vi "Receive Message.vi"(8 "error in (no error)":errorcluster, 11 "SPARC4_GEI in":refnum<class "S4GEI.lvclass">) -> (0 "error out":errorcluster, 3 "SPARC4_GEI out":refnum<class "S4GEI.lvclass">)   [LabVIEW 2018, in "S4GEI.lvclass"]
uses:
  S4GEI.lvclass
  S4GEI.lvclass/S4GEI.ctl
  Channel GUI/Channel.lvclass
  RxTx/RxTx.lvclass
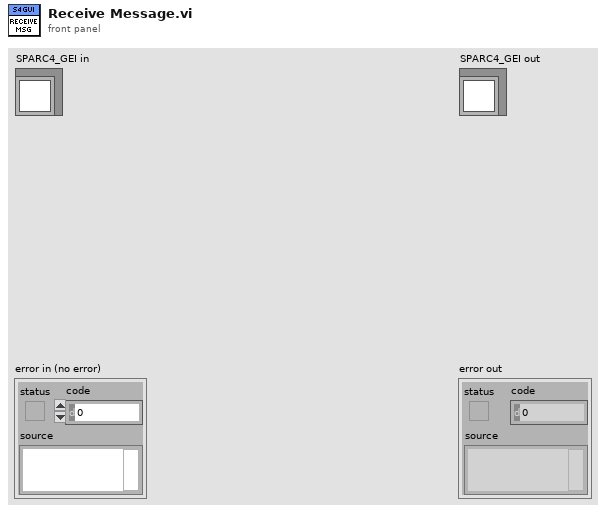
[diagram p1: front panel]
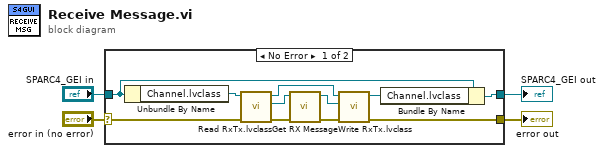
[diagram p0: block diagram]
diagram:
  n1 = case shown="No Error" "error in (no error)" {
    selector: "error in (no error)" -> [w12 w17]
    tunnel: [w10 w17] -> w3
    tunnel: [w14 w16] -> w1
    tunnel: "SPARC4_GEI in" -> [w15 w16]
    frame No Error {
      n2 = Unbundle By Name(w15) -> ("Channel.lvclass"=w13:refnum<class "Channel.lvclass">)
      n3 = call "Read RxTx.lvclass.vi"("error in (no error)"=w12, "Channel GUI in"=w13) -> ("error out"=w6:errorcluster, "RxTx.lvclass"=w9:refnum<class "RxTx.lvclass">, "Channel GUI out"=w7:refnum<class "Channel.lvclass">)  [unwired: 7 in]
      n4 = call "Get RX Message.vi"("error in (no error)"=w6, "RxTx in"=w9) -> ("error out"=w5:errorcluster, "RxTx out"=w8:refnum<class "RxTx.lvclass">)  [unwired: 7 in, 1 out]
      n5 = call "Write RxTx.lvclass.vi"("error in (no error)"=w5, "RxTx.lvclass"=w8, "Channel GUI in"=w7) -> ("error out"=w10:errorcluster, "Channel GUI out"=w11:refnum<class "Channel.lvclass">)  [unwired: 7 in]
      n6 = Bundle By Name(cluster=w15, "Channel.lvclass"=w11) -> (w14:refnum<class "S4GEI.lvclass">)
    }
    frame Error {
    }
  }
  "error out" <- w3
  "SPARC4_GEI out" <- w1
